vi "optical_1.vi"() -> ()   [LabVIEW 2025]
panel:
  out "Times between Frames":u32
  in  "STOP ACQUISITION":bool
  out "File Name Out":string
  in  "File Path":string="C:\\Digambar\\Metal_thin_wall\\Optical_images\\Optical_images"
  out "Optical Preview":T1(plugin-control)
  # "(1) Run VI"
  # "(2) After thermal camera calibration message (in terminal), press START"
  # "(3) Stop & Save"
  # "THERMAL CONTROLS"
  # "(Enter \"28\")"
  # "Thermal Record"
  # "OPTICAL CONTROLS"
  # "(must be an empty folder)"
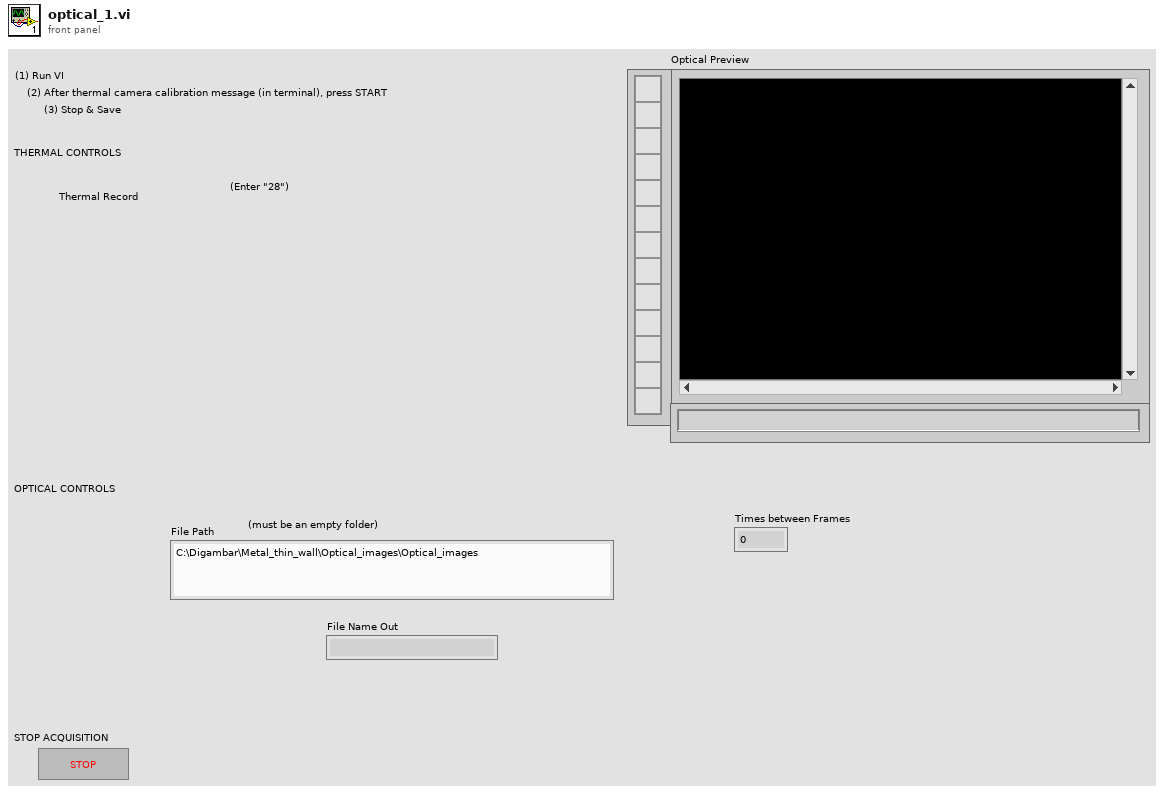
[diagram p1: front panel]
types:
  T1 = typedef "IMAQ Image.ctl" = refnum<image>
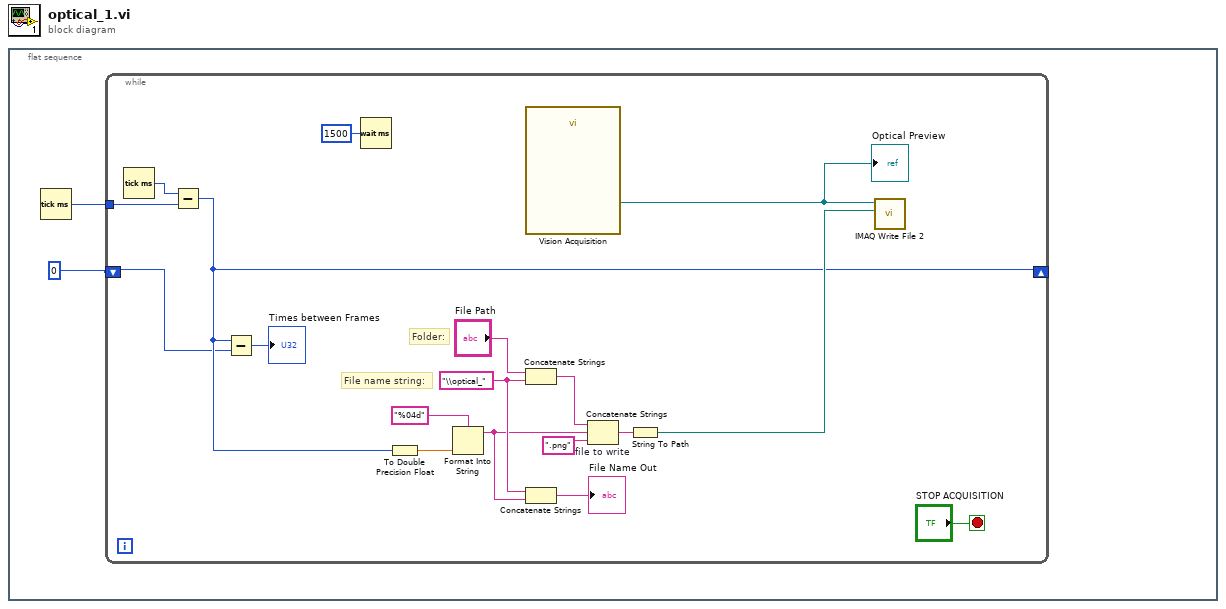
[diagram p0: block diagram]
diagram:
  n1 = flat-sequence {
    frame #0 {
      n2 = Tick Count (ms)() -> (millisecond timer value=w2:u32)
      n3 = while {
        tunnel: w2 -> [w6]
        shift-right: [w5] -> _
        shift-left: u32 0 -> [w4]
        stop <- "STOP ACQUISITION" stop-if-true
        w15 = "\\optical_" ("string")
        # "Folder:"
        # "File name string:"
        n4 = Tick Count (ms)() -> (millisecond timer value=w7:u32)
        n5 = Subtract(x=w7, y=w6) -> (x-y=w5:u32)
        n6 = Subtract(x=w5, y=w4) -> (x-y=→"Times between Frames":u32)
        n7 = Wait (ms)(milliseconds to wait=u32 1500) -> ()  [unwired: 1 out]
        n8 = To Double Precision Float(number=w5) -> (double precision float=w13:dbl)
        n9 = Format Into String(format string="%04d" ("time format string (%c)"), w13) -> (resulting string=w11:string)  [unwired: 2 in, 1 out]
        n10 = call "Vision Acquisition"() -> ("Image Out"=w20:T1)  [unwired: 26 in, 1 out]
        "Optical Preview" <- w20
        n11 = Concatenate Strings("File Path", w15) -> (w16:string)
        n12 = Concatenate Strings(w15, w11) -> (→"File Name Out":string)
        n13 = Concatenate Strings "file to write"(w16, w11, ".png" ("string")) -> (w19:string)
        n14 = String To Path(string=w19) -> (path=w12:path)
        n15 = call-poly "IMAQ Write File 2"("File Path"=w12, "Image"=w20) -> ()  [unwired: 8 in, 2 out]
      }
    }
  }
